vi "Create Getter Case in Message Handler.vi"(8 "error in (no error)":errorcluster, 11 "Getter Generator in":refnum<class "Getter Generator.lvclass">) -> (0 "error out":errorcluster, 3 "Getter Generator out":refnum<class "Getter Generator.lvclass">)   [LabVIEW 2020, in "Method Generation.lvlib" / "Getter Generator.lvclass"]
uses:
  Getter Generator.lvclass
  <vilib>/Utility/traverseref.llb/TRef TravTarget.ctl
  Getter Generator.lvclass/Getter Generator.ctl
  <vilib>/Utility/miscctls.llb/LVPointTypeDef.ctl
  <vilib>/Utility/traverseref.llb/VI Scripting - Traverse.lvlib
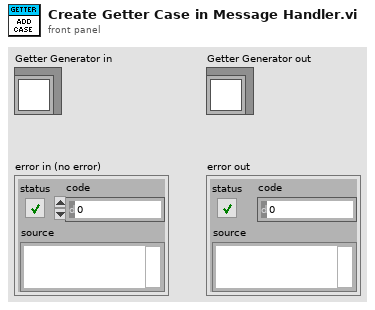
[diagram p1: front panel]
types:
  T1 = typedef "TRef TravTarget.ctl" = enum16{"FP", "BD", "Other"}
  T2 = typedef "LVPointTypeDef.ctl" = cluster{"Horizontal":i16, "Vertical":i16}
  T3 = typedef "LVBoundsTypeDef.ctl" = cluster{"Width":u32, "Height":u32}
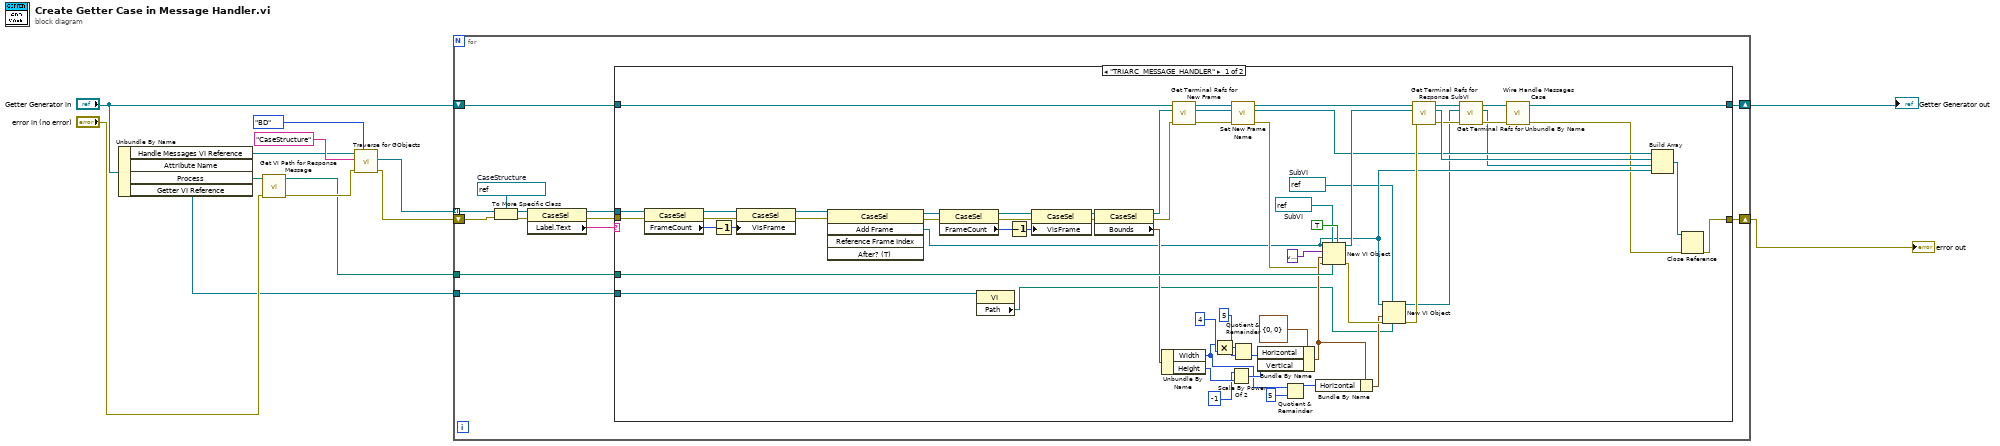
[diagram p0: block diagram]
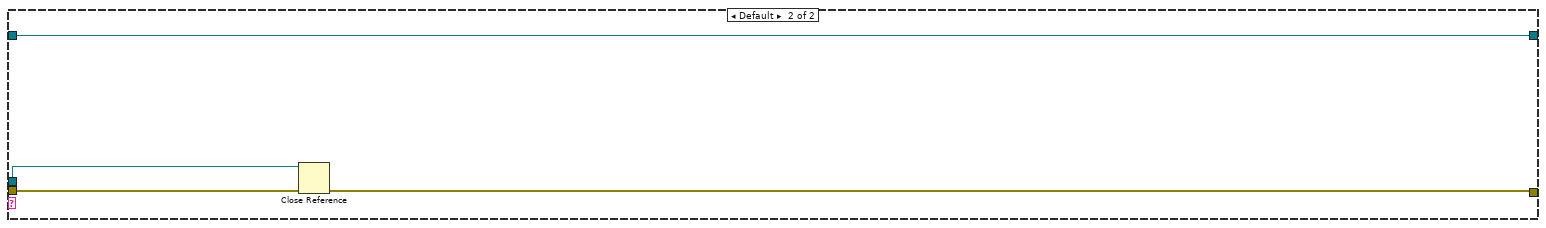
[diagram p2: hidden frame]
diagram:
  n1 = Unbundle By Name("Getter Generator in") -> ("Handle Messages VI Reference"=w3:refnum<vi>, "Process"=w11:path, "Getter VI Reference"=w1:refnum<vi>)  [unwired: 1 out]
  n2 = call "Get VI Path for Response Message.vi"("error in (no error)"="error in (no error)", "Process Path"=w11) -> ("error out"=w13:errorcluster, "Path"=w12:path)  [unwired: 8 in]
  n3 = call <vilib>:"Traverse for GObjects.vi"("Traverse Target"=TRef_TravTarget."BD", "error in (no error)"=w13, "Class Name"="CaseStructure", "VI Refnum"=w3) -> ("error out"=w4:errorcluster, "References"=w6:refnum<vi>[])  [unwired: 4 in, 2 out]
  n4 = for {
    tunnel: w6 -> [w24] mode=indexing
    shift-right: [w18] -> w5
    shift-left: w4 -> [w21]
    tunnel: w12 -> [w17]
    shift-right: [w15] -> w8
    shift-left: "Getter Generator in" -> [w16]
    tunnel: w1 -> [w14]
    w20 = refnum<vi> refnum  # CaseStructure
    n5 = To More Specific Class(target class=w20, reference=w24, error in=w21) -> (specific class reference=w23:refnum<vi>, error out=w22:errorcluster)
    n6 = property class="CaseSel"(reference=w23, error in=w22) -> (reference out=w25:refnum<vi>, error out=w19:errorcluster, "Label.Text"=w26:string)
    n7 = case shown="\"TRIARC_MESSAGE_HANDLER\"" w26 {
      tunnel: w25 -> [w27 w91]
      tunnel: w19 -> [w29 w90]
      tunnel: [w61 w89] -> w18
      tunnel: w17 -> [w84 _]
      tunnel: w16 -> [w68 w88]
      tunnel: [w58 w88] -> w15
      tunnel: w14 -> [w39 _]
      frame "TRIARC_MESSAGE_HANDLER" {
        w40 = refnum<vi> refnum  # SubVI
        w86 = refnum<vi> refnum  # SubVI
        n8 = property class="CaseSel"(reference=w27, error in=w29) -> (reference out=w32:refnum<vi>, error out=w33:errorcluster, "FrameCount"=w31:i32)
        n9 = Decrement(x=w31) -> (x-1=w34:i32)
        n10 = property class="CaseSel"(reference=w32, error in=w33, "VisFrame"=w34) -> (reference out=w28:refnum<vi>, error out=w30:errorcluster)
        n11 = invoke class="CaseSel" method="Add Frame"(reference=w28, error in=w30) -> (reference out=w47:refnum<vi>, error out=w43:errorcluster, "Add Frame"=w49:refnum<vi>)  [unwired: 3 in, 2 out]
        n12 = property class="CaseSel"(reference=w47, error in=w43) -> (reference out=w46:refnum<vi>, error out=w44:errorcluster, "FrameCount"=w48:i32)
        n13 = property class="VI"(reference=w39) -> ("Path"=w38:path)  [unwired: 1 in, 2 out]
        n14 = Decrement(x=w48) -> (x-1=w41:i32)
        n15 = property class="CaseSel"(reference=w46, error in=w44, "VisFrame"=w41) -> (reference out=w45:refnum<vi>, error out=w42:errorcluster)
        n16 = property class="CaseSel"(reference=w45, error in=w42) -> (reference out=w67:refnum<vi>, error out=w66:errorcluster, "Bounds"=w78:T3)
        n17 = Unbundle By Name(w78) -> ("Width"=w72:u32, "Height"=w83:u32)
        n18 = call "Get Terminal Refs for New Frame.vi"("error in (no error)"=w66, "Case Structure Ref"=w67, "Getter Generator In"=w68) -> ("error out"=w52:errorcluster, "reference out"=w54:refnum<vi>, "Getter Generator Out"=w64:refnum<class "Getter Generator.lvclass">)  [unwired: 6 in]
        n19 = Multiply(x=w72, y=u32 4) -> (x*y=w76:u32)
        n20 = Scale By Power Of 2(n=i16 -1, x=w83) -> (x*2^n=w80:u32)
        n21 = call "Set New Frame Name.vi"("error in (no error)"=w52, "reference in"=w54, "Getter Generator in"=w64) -> ("error out"=w51:errorcluster, "reference out"=w53:refnum<vi>, "Getter Generator out"=w50:refnum<class "Getter Generator.lvclass">)  [unwired: 6 in]
        n22 = Quotient & Remainder(x=w76, y=u32 5) -> (floor(x/y)=w81:u32)  [unwired: 1 out]
        n23 = Bundle By Name(cluster=T2 {"Horizontal"=0, "Vertical"=0} ("location"), "Horizontal"=w81, "Vertical"=w80) -> (w73:T2)
        n24 = Quotient & Remainder(x=w72, y=u32 5) -> (floor(x/y)=w70:u32)  [unwired: 1 out]
        n25 = Bundle By Name(cluster=w73, "Horizontal"=w70) -> (w69:T2)
        n26 = New VI Object(vi object class=w86, auto wire? (F)=TRUE, owner refnum=w49, style=variant, position/next to=w73, 6:w84, 8:w51) -> (object refnum=w65:refnum<vi>, 0:w74:errorcluster)  [unwired: 1 in]
        n27 = New VI Object(vi object class=w40, owner refnum=w49, position/next to=w69, 6:w38, 8:w74) -> (object refnum=w35:refnum<vi>, 0:w55:errorcluster)  [unwired: 3 in]
        n28 = call "Get Terminal Refs for Response SubVI.vi"("error in (no error)"=w55, "object refnum"=w65, "Getter Generator In"=w50) -> ("error out"=w57:errorcluster, "reference out"=w62:refnum<vi>, "Getter Generator Out"=w60:refnum<class "Getter Generator.lvclass">)  [unwired: 6 in]
        n29 = call "Get Terminal Refs for Unbundle By Name.vi"("error in (no error)"=w57, "SubVI ref"=w35, "Getter Generator In"=w60) -> ("error out"=w56:errorcluster, "SubVI ref out"=w37:refnum<vi>, "Getter Generator Out"=w59:refnum<class "Getter Generator.lvclass">)  [unwired: 6 in]
        n30 = call "Wire Handle Messages Case.vi"("error in (no error)"=w56, "Getter Generator in"=w59) -> ("error out"=w36:errorcluster, "Getter Generator out"=w58:refnum<class "Getter Generator.lvclass">)  [unwired: 8 in]
        n31 = Build Array(w53, w62, w37, w49) -> (w63:refnum<vi>[])
        n32 = Close Reference(reference=w63, error in (no error)=w36) -> (error out=w61:errorcluster)
      }
      frame Default {
        n33 = Close Reference(reference=w91, error in (no error)=w90) -> (error out=w89:errorcluster)
      }
    }
  }
  "Getter Generator out" <- w8
  "error out" <- w5
